vi "Header Astep.vi"(8 "日付/時間文字列":string, 11 "文字列":string) -> (3 "Header for Astep":string)   [LabVIEW 2018]
panel:
  out "数字の部分 2":string
  out "部分文字列の前 2":string
  out "部分文字列の前":string
  out "部分文字列の後":string
  out "数字の部分":string
  out "Ex Name Part":string
  # "OM1-03_1st#003 D_20180207_1922 TOAN#1Pex4n1_OM1-03_1st_EXSV#1_20180207_1959_SGM  D0.580nm B100vsI_8.86_EP1_100_EP2_-101.tdms"
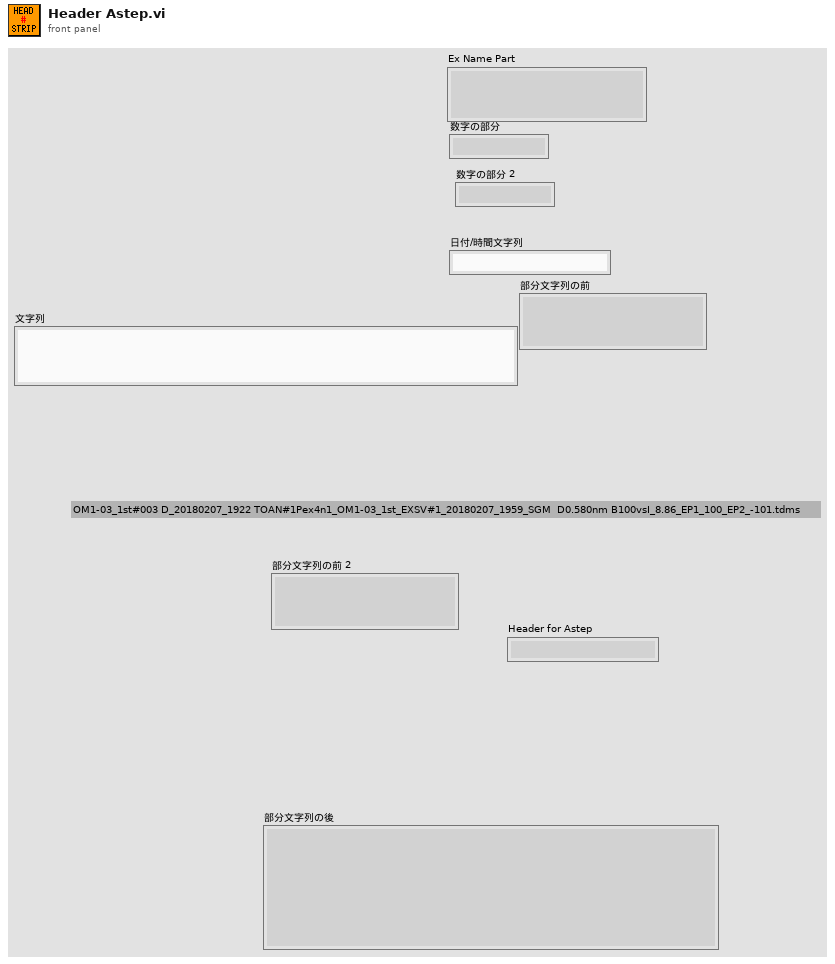
[diagram p1: front panel]
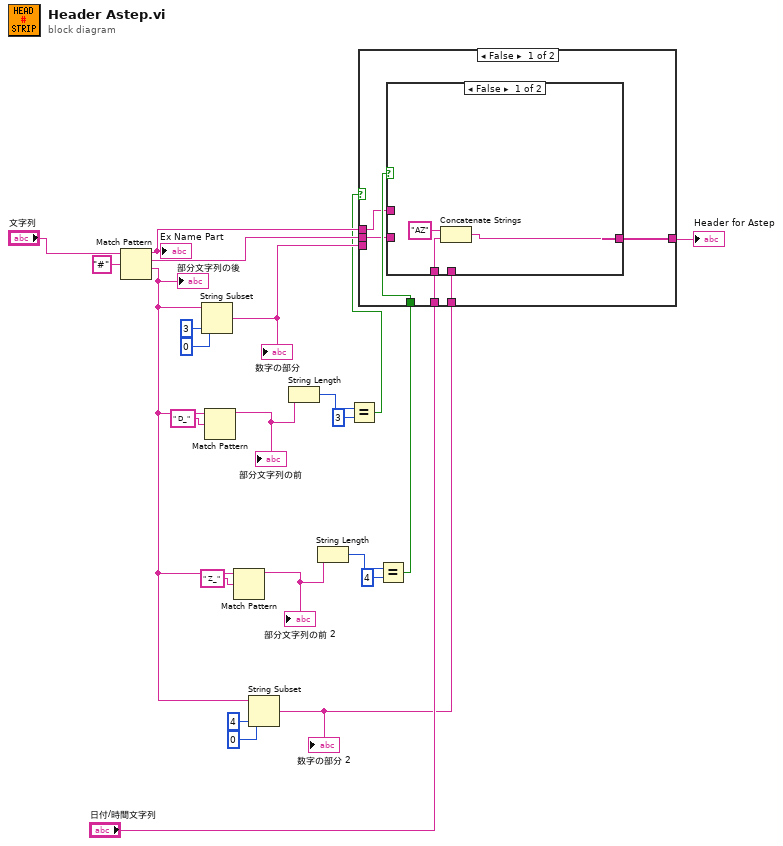
[diagram p0: block diagram]
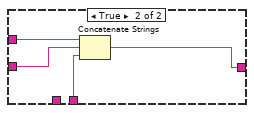
[diagram p2: hidden frame]
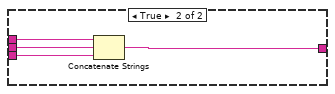
[diagram p3: hidden frame]
diagram:
  n1 = Match Pattern(string="文字列", regular expression="#" ("正規表現")) -> (before substring=w19:string, match substring=w18:string, after substring=w4:string)  [unwired: 1 in, 1 out]
  "Ex Name Part" <- w19
  "部分文字列の後" <- w4
  n2 = String Subset(string=w4, offset (0)=0 ("オフセット（0）"), length (rest)=3 ("長さ（残り）")) -> (substring=w16:string)
  "数字の部分" <- w16
  n3 = Match Pattern(string=w4, regular expression=" D_" ("検索文字列")) -> (before substring=w2:string)  [unwired: 1 in, 3 out]
  "部分文字列の前" <- w2
  n4 = Match Pattern(string=w4, regular expression=" Z_" ("検索文字列")) -> (before substring=w1:string)  [unwired: 1 in, 3 out]
  "部分文字列の前 2" <- w1
  n5 = String Subset(string=w4, offset (0)=0 ("オフセット（0）"), length (rest)=4 ("長さ（残り）")) -> (substring=w3:string)
  "数字の部分 2" <- w3
  n6 = String Length(string=w2) -> (length=w15:i32)
  n7 = String Length(string=w1) -> (length=w10:i32)
  n8 = Equal?(x=w15, y=3) -> (x = y?=w13:bool)
  n9 = Equal?(x=w10, y=4) -> (x = y?=w7:bool)
  n10 = case shown="False" w13 {
    tunnel: w19 -> [w26 w40]
    tunnel: w18 -> [w25 w39]
    tunnel: [w29 w38] -> w17
    tunnel: w16 -> [_ w37]
    tunnel: "日付/時間文字列" -> [w28 _]
    tunnel: w7 -> [w27 _]
    tunnel: w3 -> [w24 _]
    frame False {
      n11 = case shown="False" w27 {
        tunnel: [w32 w33] -> w29
        tunnel: w28 -> [w31 _]
        tunnel: w26 -> [_ w36]
        tunnel: w25 -> [_ w34]
        tunnel: w24 -> [_ w35]
        frame False {
          n12 = Concatenate Strings("AZ" ("文字列"), w31) -> (w32:string)
        }
        frame True {
          n13 = Concatenate Strings(w36, w34, w35) -> (w33:string)
        }
      }
    }
    frame True {
      n14 = Concatenate Strings(w40, w39, w37) -> (w38:string)
    }
  }
  "Header for Astep" <- w17
